vi "Probador.vi"() -> ()   [LabVIEW 2026]
panel:
  in  "Combo Box":string(combo)
  in  "Test":bool
  in  "Stop Button":bool
  out "unsigned byte array":u8[](array[numeric]) format="%x"
  out "error out":errorcluster
  out "respuesta":string
  in  "Comando":u8[](array[numeric]) format="%x"
  in  "VISA resource name":refnum<visa-resource-name>
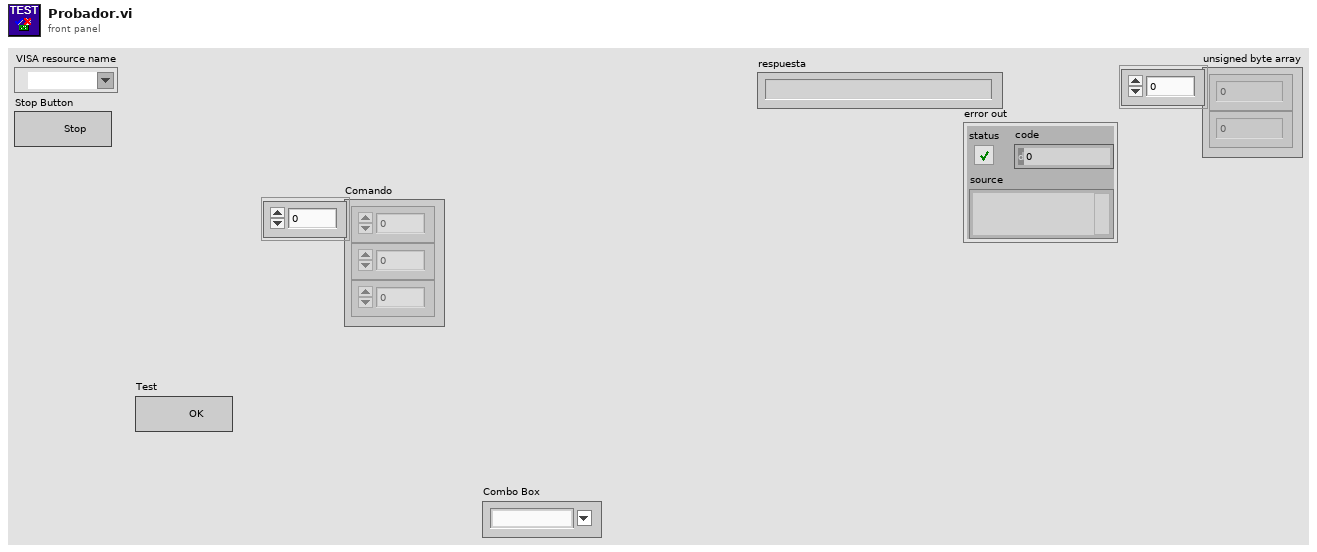
[diagram p1: front panel]
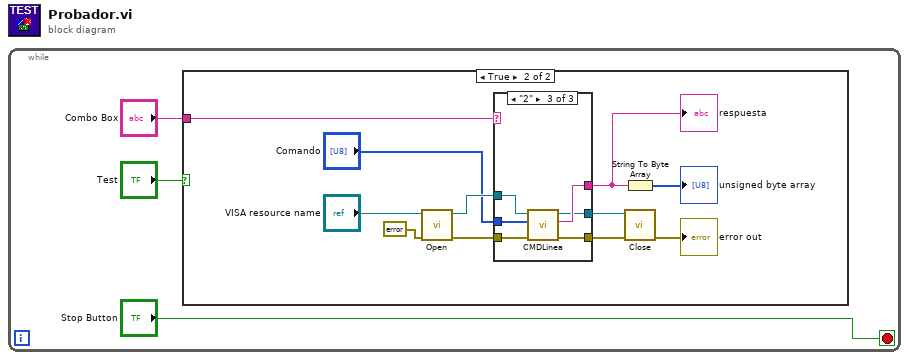
[diagram p0: block diagram]
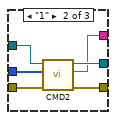
[diagram p4: hidden frame]
diagram:
  n1 = while {
    stop <- "Stop Button" stop-if-true
    n2 = case shown="True" "Test" {
      tunnel: "Combo Box" -> [_ w4]
      frame False {
      }
      frame True {
        n3 = call "Open.vi"("error in (no error)"=errorcluster {"status"=FALSE, "code"=0, "source"=""}, "VISA resource name"="VISA resource name") -> ("error out"=w12:errorcluster, "VISA resource name out"=w9:refnum<visa-resource-name>)  [unwired: 8 in]
        n4 = case shown="\"2\"" w4 {
          tunnel: w12 -> [_ w20 w24]
          tunnel: [_ w19 w23] -> w11
          tunnel: [_ w18 w21] -> w10
          tunnel: w9 -> [_ w17 w26]
          tunnel: "Comando" -> [_ w16 w25]
          tunnel: [_ w15 w22] -> w6
          frame "False", Default {
          }
          frame "1" {
            n5 = call "CMD2.vi"("error in (no error)"=w20, "Comando"=w16, "VISA resource name"=w17) -> ("error out"=w19:errorcluster, "respuesta"=w15:string, "VISA resource name out"=w18:refnum<visa-resource-name>)  [unwired: 6 in]
          }
          frame "2" {
            n6 = call "CMDLinea.vi"("error in (no error)"=w24, "Comando"=w25, "VISA resource name"=w26) -> ("error out"=w23:errorcluster, "respuesta"=w22:string, "VISA resource name out"=w21:refnum<visa-resource-name>)  [unwired: 6 in]
          }
        }
        "respuesta" <- w6
        n7 = String To Byte Array(string=w6) -> (unsigned byte array=→"unsigned byte array":u8[])
        n8 = call "Close.vi"("error in (no error)"=w11, "VISA resource name"=w10) -> ("error out"=→"error out":errorcluster)  [unwired: 9 in]
      }
    }
  }
